vi "Handle Activation.vi"(8 "error in (no error)":errorcluster, 10 "Activation":T1, 11 "ActivationHandler in":refnum<class "ActivationHandler.lvclass">) -> ()   [LabVIEW 2026, in "ToastNotification.lvlib" / "ActivationHandler.lvclass"]
doc: "Dynamic-dispatch extension point for an injected activation handler. Override this method in a child class to process Activation.Arguments and Activation.User Inputs. The current base implementation performs no action and propagates the incoming error; it displays no dialog. Protocol-activation buttons are handled by Windows rather than this method. Application handlers should return promptly and send long-running work to a caller-owned queue or user event. Never close the service from its callback."
uses:
  ActivationHandler.lvclass
  ToastNotification/Activation.ctl
  ToastNotification/Argument.ctl
  ToastNotification/ToastNotification.lvlib
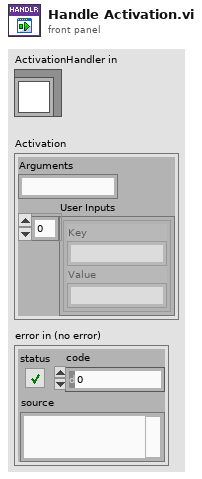
[diagram p1: front panel]
types:
  T1 = typedef "ToastNotification.lvlib/Activation.ctl" = cluster{"Arguments":string, "User Inputs":T2[]}
  T2 = typedef "ToastNotification.lvlib/Argument.ctl" = cluster{"Key":string, "Value":string}
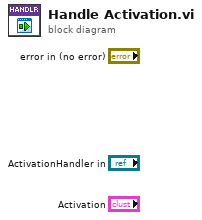
[diagram p0: block diagram]
diagram:
